vi "engine mappings UI.vi"() -> ()   [LabVIEW 2014, in "PL Framework Configuration Tool.lvlib" / "Engine Mappings.lvclass"]
uses:
  Engine Mappings.lvclass
  <vilib>/NI/Configuration Framework/Node/NodeRef.ctl
  <vilib>/NI/Configuration Framework/Node/NISE_CEF_Node.lvclass
  <vilib>/NI/AMC/Message Queue.ctl
  <vilib>/NI/AMC/Message.ctl
  <vilib>/NI/Tools/Keyed Array/KeyedArray.ctl
  <vilib>/NI/Configuration Framework/Node/UserEventRef.ctl
  <vilib>/NI/Configuration Framework/Controls/EventCluster.ctl
  <vilib>/NI/DCAF UI Toolkit/Controls/Move One Right.ctl
  <vilib>/NI/DCAF UI Toolkit/Controls/Move One Left.ctl
  <vilib>/NI/DCAF UI Toolkit/Controls/Export.ctl
  <vilib>/NI/Configuration Framework/Node/RefreshUIEvent.ctl
  <vilib>/NI/Configuration Framework/Node/CacheState.ctl
  <vilib>/NI/Configuration Framework/Node/StopEvent.ctl
  <vilib>/NI/Configuration Framework/Node/NodeChangeEvent.ctl
  subVIs/Mapping.ctl
  <vilib>/Utility/miscctls.llb/LVPositionTypeDef.ctl
  <vilib>/NI/Configuration Framework/serializable configuration/NISE_CEF_serializable configuration.lvclass/NISE_CEF_serializable configuration.ctl
  <vilib>/NI/Tag Bus/tag/tag descriptor.lvclass/tag descriptor.ctl
  <vilib>/NI/Tag Bus Module Framework/channel/channel classification.ctl
  <vilib>/NI/Configuration Framework/serializable configuration/get alias.vi
  <vilib>/Utility/LVClass/Get LV Class Name.vi
  <vilib>/NI/Configuration Framework/error generator/NISE_error generator.vi
  <vilib>/NI/Tag Bus Module Framework/module configuration/TBM module configuration.lvclass
  <vilib>/NI/Module Execution Interface/Engine Configuration/engine configuration.lvclass
  <vilib>/NI/Tag Bus/tag/tag descriptor.lvclass
  Engine Parent/Engine Parent Editor Node.lvclass
  Robust CSV/Robust CSV.lvlib
  <vilib>/NI/Configuration Framework/serializable configuration/NISE_CEF_serializable configuration.lvclass
  <vilib>/NI/Tag Bus Module Framework/channel/TBM channel.lvclass
  Utilities/GraphViz Vizualizations/GraphViz Mapping Visualizer.lvlib
  <vilib>/NI/DCAF UI Toolkit/Controls/DCAF UI Elements.lvlib
  <vilib>/NI/Tools/Keyed Array/Tools_KeyedArray.lvlib
  <vilib>/NI/AMC/AMC.lvlib
  <vilib>/NI/Configuration Framework/NISE_CEF_TreeControl.lvlib
panel:
  in  "Tab Control":T1(tab)
  in  "Show Mappings":T2
  in  "channels":i32(listbox)
  in  "Tags":i32(listbox)
  in  "map":T3
  in  "unmap":T4
  in  "export CSV":T5
  in  "Mappings":i32(listbox)
  out "Writer Channel":string
  out "channels reading tag to outout":i32(listbox)
  out "channels from input":i32(listbox)
  in  "outputs":i32(listbox)
  in  "method selection":enum32{"Inputs and Outputs", "Processing"}(radio)
  in  "inputs":i32(listbox)
  in  "Module to View":u16(ring)
  in  "attempt mapping":bool
  in  "Module 1 Filter":string
  in  "Module 2 Filter":string
  in  "Module 2 Channels":i32[](listbox)
  in  "Module 1 Channels":i32[](listbox)
  in  "Module 2":u16(ring)
  in  "Module 1":u16(ring)
  in  "main queue":T6
  in  "node ref":T7
  in  "user event":T8
  in  "node change":T9
  in  "stop event":T10
  in  "cache state":T11
  in  "refresh UI":T12
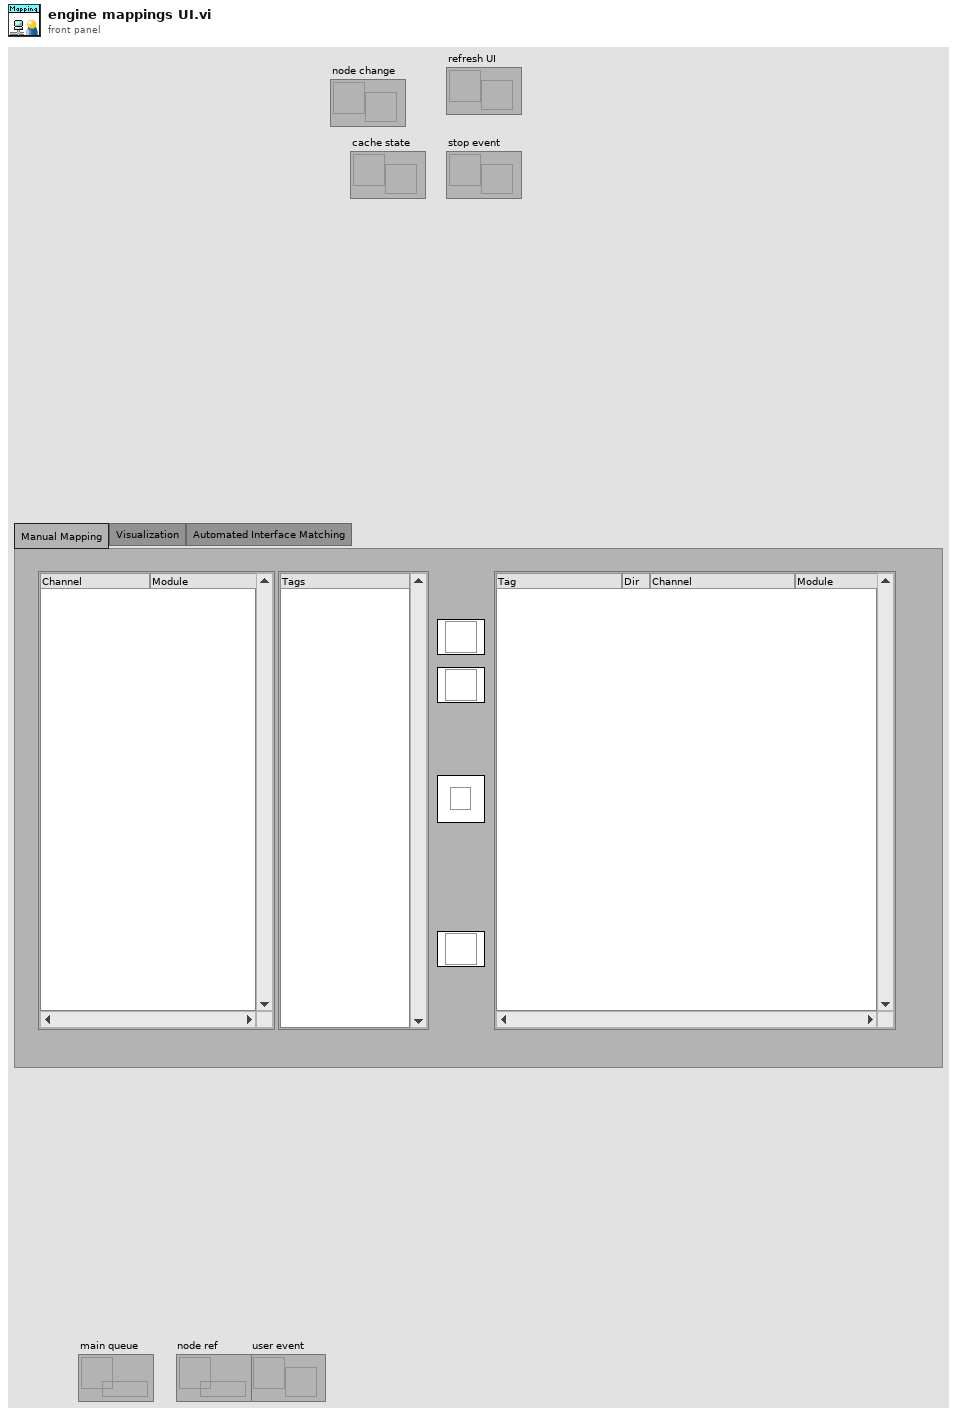
[diagram p1: front panel]
types:
  T1 = enum32{"Manual Mapping", "Visualization", "Automated Interface Matching"}
  T2 = typedef "Mapping.ctl" = bool
  T3 = typedef "DCAF UI Elements.lvlib/Move One Right.ctl" = bool
  T4 = typedef "DCAF UI Elements.lvlib/Move One Left.ctl" = bool
  T5 = typedef "DCAF UI Elements.lvlib/Export.ctl" = bool
  T6 = typedef "AMC.lvlib/Message Queue.ctl" = refnum<queue>
  T7 = typedef "NISE_CEF_Node.lvclass/NodeRef.ctl" = refnum<data-value>
  T8 = typedef "NISE_CEF_Node.lvclass/UserEventRef.ctl" = refnum<user-event>
  T9 = typedef "NISE_CEF_Node.lvclass/NodeChangeEvent.ctl" = refnum<user-event>
  T10 = typedef "NISE_CEF_Node.lvclass/StopEvent.ctl" = refnum<user-event>
  T11 = typedef "NISE_CEF_Node.lvclass/CacheState.ctl" = refnum<user-event>
  T12 = typedef "NISE_CEF_Node.lvclass/RefreshUIEvent.ctl" = refnum<user-event>
  T13 = typedef "LVPositionTypeDef.ctl" = cluster{"Left":i32, "Top":i32}
  T14 = typedef "TBM channel.lvclass/channel classification.ctl" = enum16{"input data", "output data", "processing parameter", "processing result"}
  T15 = typedef "engine configuration.lvclass/unique channel identifier.ctl" = cluster{"channel":string, "module ID":string}
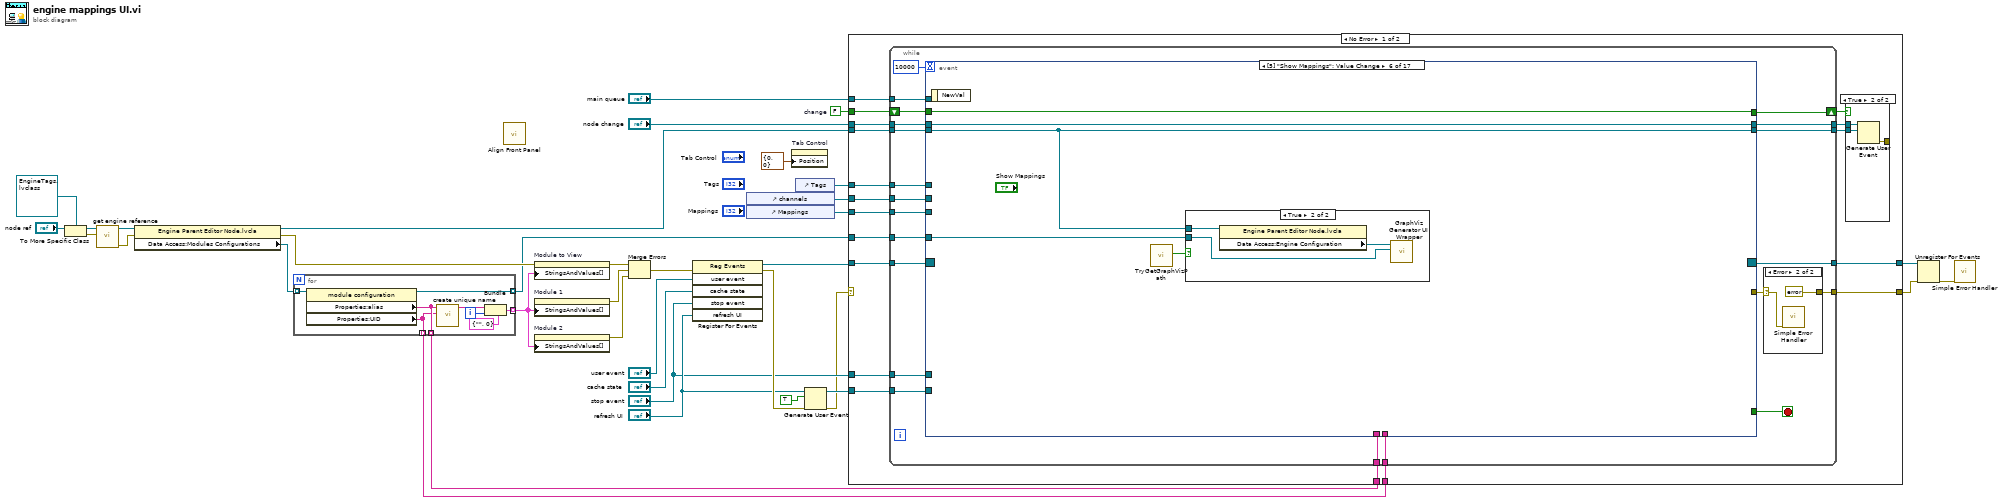
[diagram p0: block diagram]
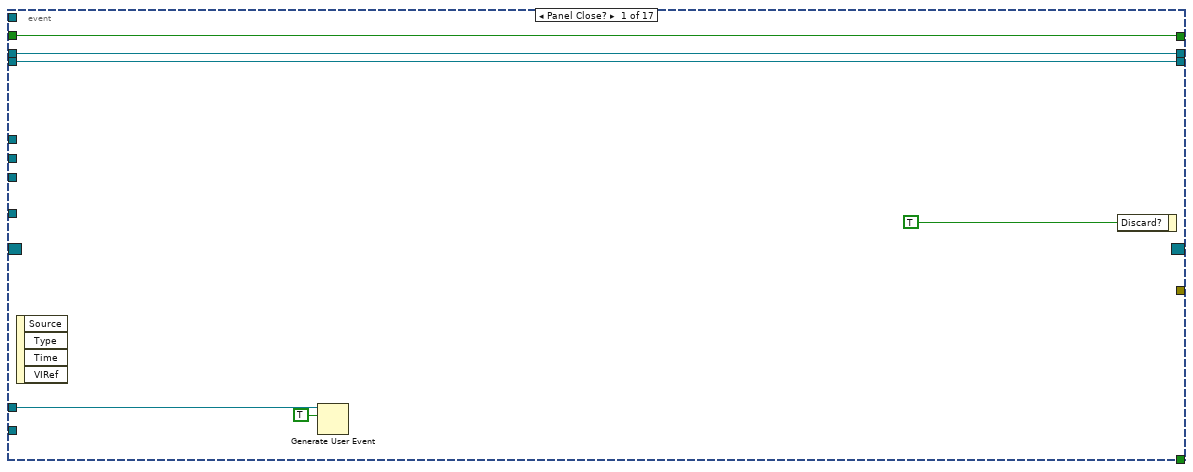
[diagram p4: hidden frame]
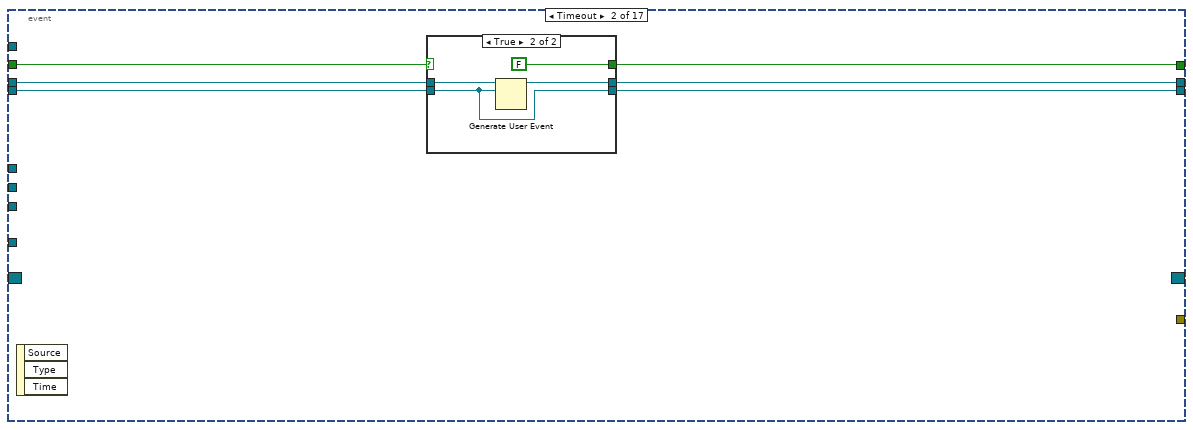
[diagram p5: hidden frame]
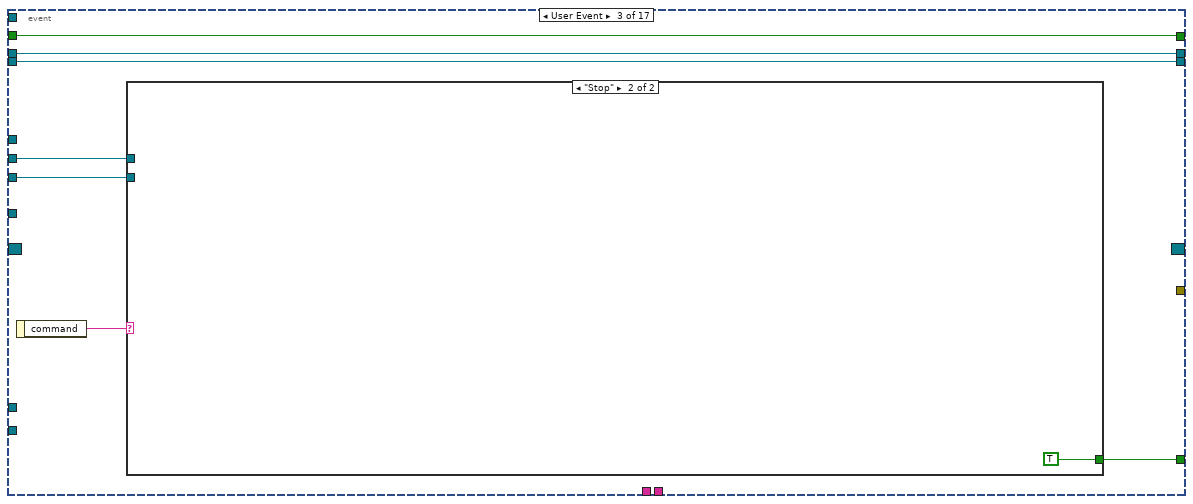
[diagram p7: hidden frame]
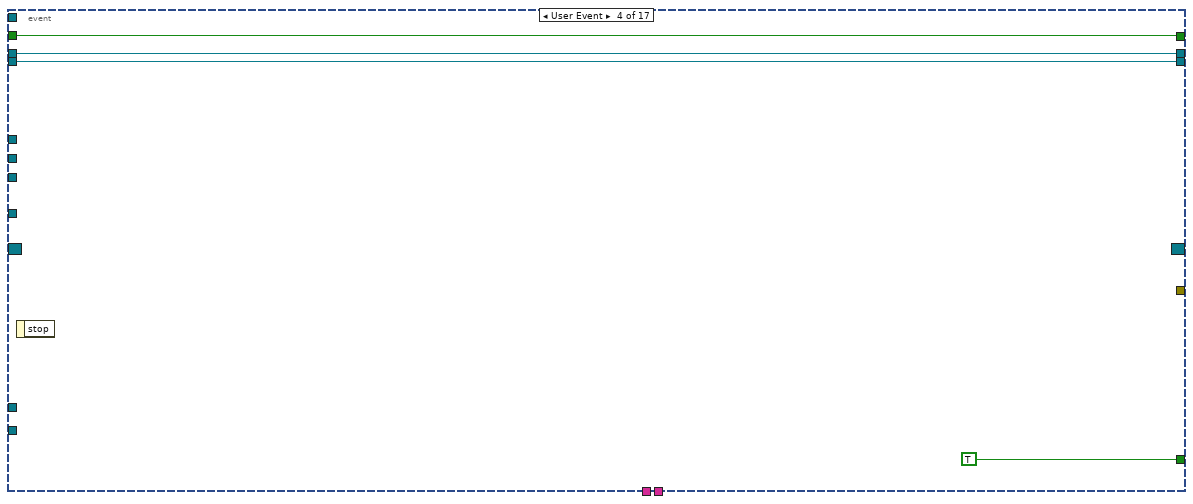
[diagram p9: hidden frame]
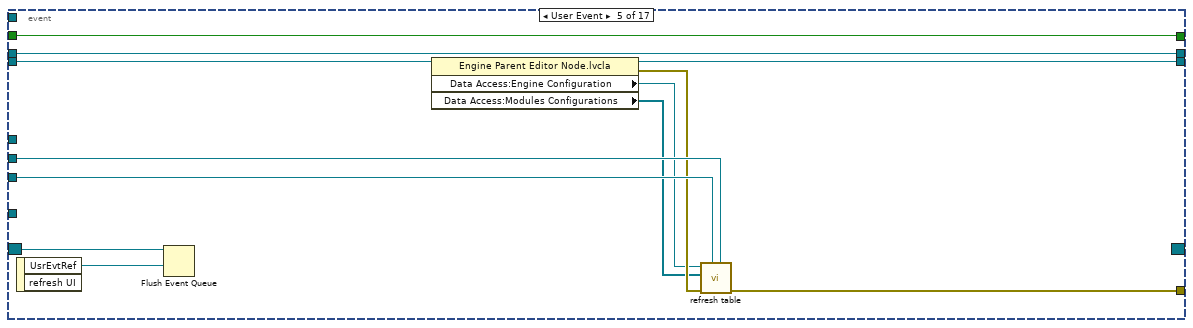
[diagram p10: hidden frame]
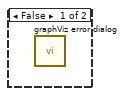
[diagram p11: hidden frame]
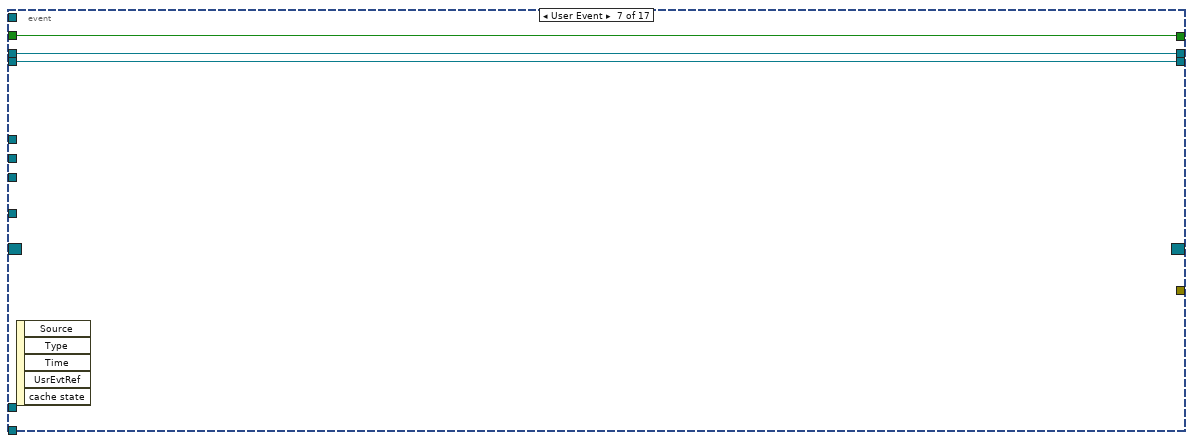
[diagram p12: hidden frame]
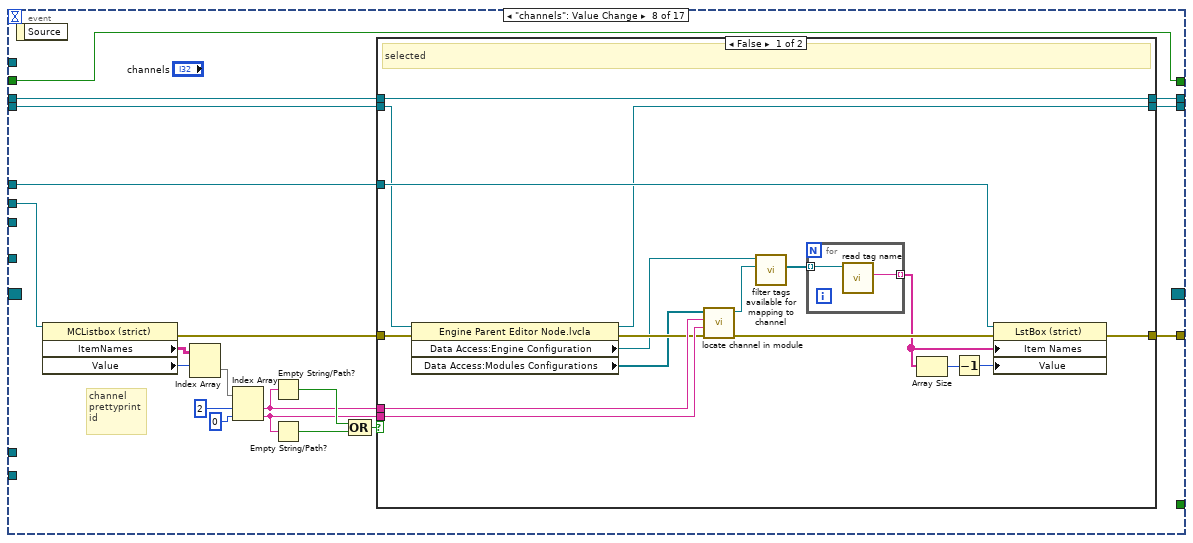
[diagram p13: hidden frame]
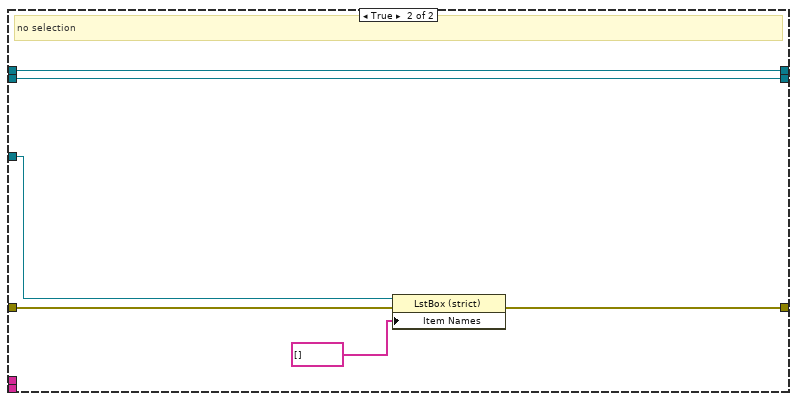
[diagram p14: hidden frame]
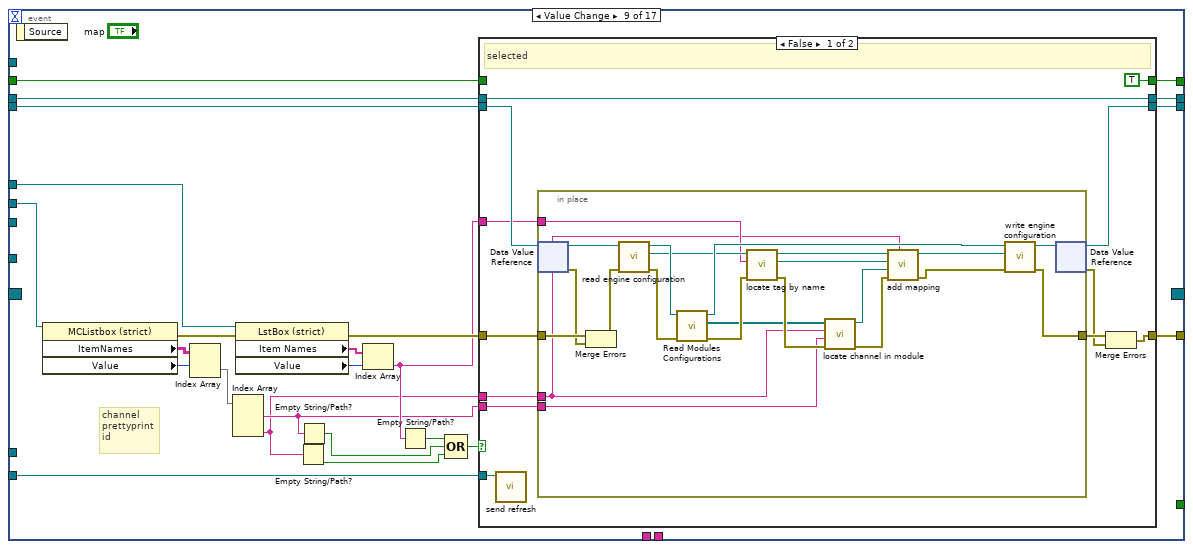
[diagram p15: hidden frame]
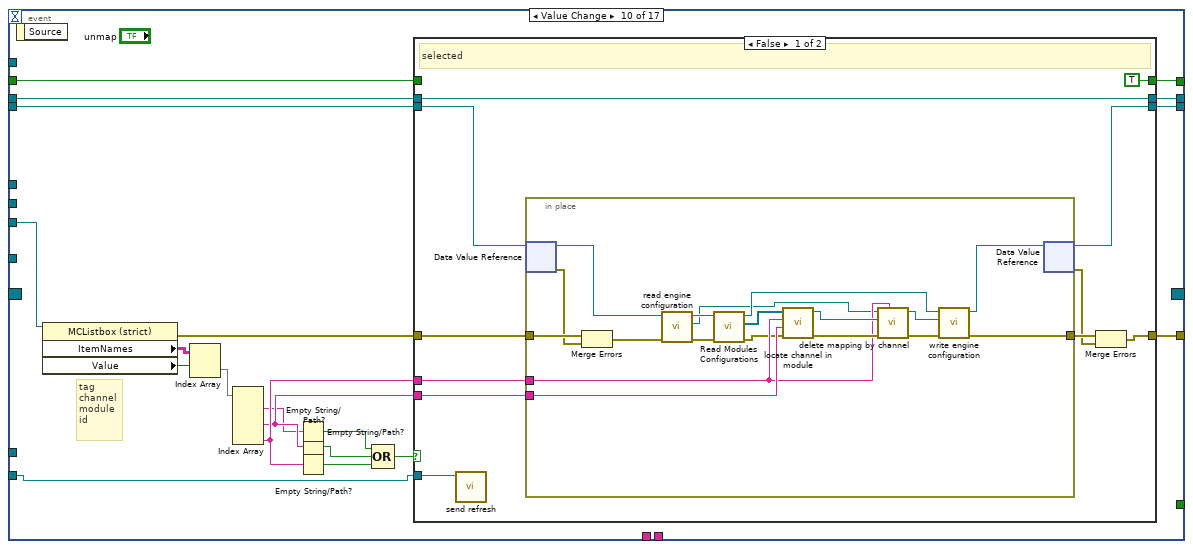
[diagram p17: hidden frame]
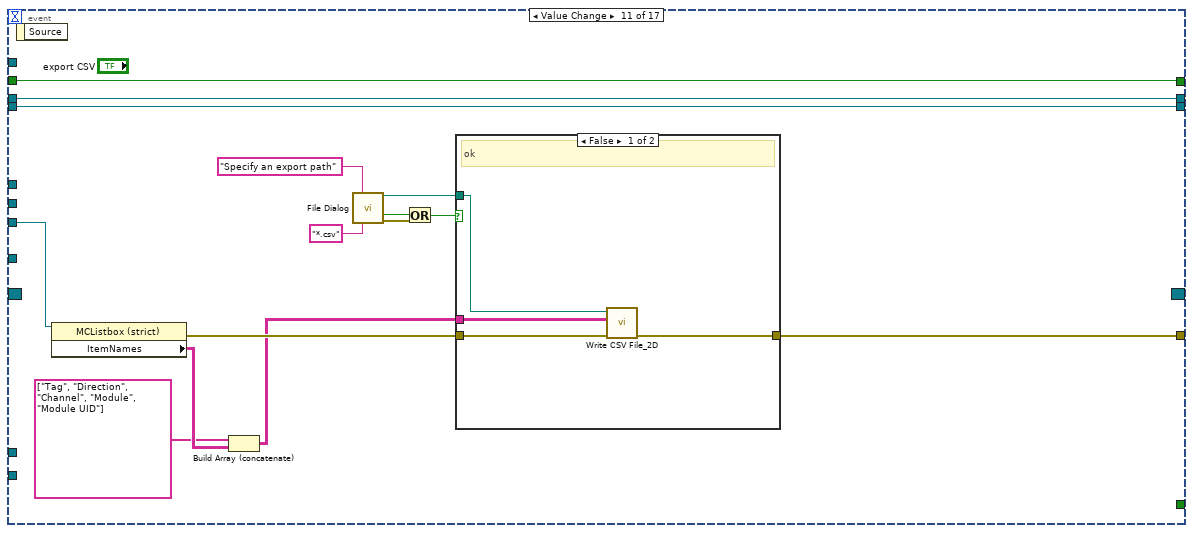
[diagram p19: hidden frame]
diagram:
  w1 = FALSE  # change
  n1 = To More Specific Class(target class=refnum<data-value> refnum ("data value reference"), reference="node ref") -> (specific class reference=w22:refnum<data-value>, error out=w23:errorcluster)  [unwired: 1 in]
  n2 = call "get engine reference.vi"("error in"=w23, "engine mappings"=w22) -> ("error out"=w25:errorcluster, "engine reference"=w17:refnum<data-value>)  [unwired: 8 in]
  n3 = property class="Engine Parent Editor Node.lvcla"(reference=w17, error in=w25) -> (reference out=w16:refnum<data-value>, error out=w15:errorcluster, "Data Access:Modules Configurations"=w14:refnum<class "TBM module configuration.lvclass">[])
  n4 = for {
    tunnel: w14 -> [w44] mode=indexing
    tunnel: [w43] -> w13 mode=indexing
    tunnel: [w42] -> w12 mode=indexing
    tunnel: [w40] -> w11 mode=indexing
    tunnel: [w37] -> w2 mode=indexing
    i -> [w38]
    n5 = property class="module configuration"(reference=w44) -> (reference out=w37:refnum<class "TBM module configuration.lvclass">, "Properties:alias"=w43:string, "Properties:UID"=w42:string)  [unwired: 1 in, 1 out]
    n6 = call "create unique name.vi"("UID"=w42, "alias"=w43) -> ("unique ring name"=w39:string)  [unwired: 9 in]
    n7 = Bundle(cluster=cluster{"String":string, "Value":u16} {"String"="", "Value"=0}, "String"=w39, "Value"=w38) -> (w40:cluster{"String":string, "Value":u16})
  }
  n8 = call <vilib>:"Align Front Panel.vi"() -> ()  [unwired: 10 in, 2 out]
  n9 = property on="Module to View" class="Ring (strict)"(error in=w15, "StringsAndValues[]"=w11) -> (error out=w8:errorcluster)  [unwired: 1 in, 1 out]
  n10 = property on="Module 1" class="Ring (strict)"("StringsAndValues[]"=w11) -> (error out=w7:errorcluster)  [unwired: 2 in, 1 out]
  n11 = property on="Module 2" class="Ring (strict)"("StringsAndValues[]"=w11) -> (error out=w6:errorcluster)  [unwired: 2 in, 1 out]
  n12 = Merge Errors(w8, w7, w6) -> (w5:errorcluster)
  n13 = register-events(error in=w5, "user event", "cache state", "stop event", "refresh UI") -> (reference out=w35:refnum<event-registration>, error out=w32:errorcluster)  [unwired: 1 in]
  n14 = control-ref of="channels"() -> (w27:refnum<vi>)
  n15 = control-ref of="Mappings"() -> (w26:refnum<vi>)
  n16 = property on="Tab Control" class="TabCtl (strict)"("Position"=T13 {"Left"=0, "Top"=0}) -> ()  [unwired: 2 in, 2 out]
  n17 = control-ref of="Tags"() -> (w28:refnum<vi>)
  n18 = Generate User Event(user event="refresh UI", event data cluster=TRUE ("event data"), error in=w32) -> (user event out=w29:T12, error out=w4:errorcluster)  [unwired: 1 in]
  n19 = case shown="No Error" w4 {
    selector: w4 -> [_ w653]
    tunnel: "main queue" -> [w62 _]
    tunnel: w35 -> [w61 w654]
    tunnel: [w60 w654] -> w34
    tunnel: [w59 w653] -> w33
    tunnel: w16 -> [w48 _]
    tunnel: w29 -> [w58 _]
    tunnel: w28 -> [w57 _]
    tunnel: w27 -> [w56 _]
    tunnel: w26 -> [w55 _]
    tunnel: "stop event" -> [w54 _]
    tunnel: "node change" -> [w52 _]
    tunnel: w2 -> [w51 _]
    tunnel: w13 -> [w50 _]
    tunnel: w12 -> [w49 _]
    tunnel: w1 -> [w45 _]
    frame No Error {
      n20 = while {
        tunnel: w62 -> [w86]
        tunnel: w61 -> [w85]
        tunnel: [w84] -> w60
        tunnel: w48 -> [w81]
        tunnel: w58 -> [w79]
        tunnel: w57 -> [w78]
        tunnel: w56 -> [w77]
        tunnel: w55 -> [w76]
        tunnel: w54 -> [w75]
        tunnel: [w82] -> w59
        shift-right: [w73] -> w53
        shift-left: w45 -> [w74]
        tunnel: w52 -> [w71]
        tunnel: w51 -> [w70]
        tunnel: w50 -> [w69]
        tunnel: w49 -> [w68]
        tunnel: [w67] -> w47
        tunnel: [w66] -> w46
        stop <- w83 stop-if-true
        n21 = event shown="[5] \"Show Mappings\": Value Change" {
          selector: w85 -> [_ _ _ _ w125 _ _ _ _ _ _ _ _ _ _ _ _]
          dyn-events: [_ _ _ _ _ _ _ _ _ _ _ _ _ _ _ _ _] -> w84
          timeout: 10000 -> [_ _ _ _ _ _ _ _ _ _ _ _ _ _ _ _ _]
          tunnel: w86 -> [_ _ _ _ _ _ _ _ _ _ _ _ _ _ _ _ _]
          tunnel: [_ _ w115 TRUE _ _ _ _ _ _ _ _ _ _ _ _ _] -> w83
          tunnel: [_ _ _ _ w132 _ _ w154 w198 w263 w308 _ w385 w448 w515 w539 w560] -> w80
          tunnel: w81 -> [w90 w97 w109 w117 w122 w135 w141 w151 w193 w255 w303 w324 w388 w451 w512 w535 w561]
          tunnel: w79 -> [_ _ _ _ _ _ _ _ w197 w262 _ _ _ _ _ _ _]
          tunnel: w78 -> [_ _ _ _ _ _ _ w152 w211 _ _ _ _ _ _ _ _]
          tunnel: w77 -> [_ _ w113 _ w131 _ _ w161 w209 _ _ _ _ _ _ _ _]
          tunnel: w76 -> [_ _ w112 _ w130 _ _ _ _ w261 w317 _ _ _ _ _ _]
          tunnel: w75 -> [w94 _ _ _ _ _ _ _ _ _ _ _ _ _ _ _ _]
          tunnel: w74 -> [w92 w101 w111 w119 w126 w137 w143 w150 w192 w253 w305 w335 w403 w465 w525 w548 w558]
          tunnel: [w92 w100 w111 w119 w126 w137 w143 w150 w191 w254 w305 w335 w403 w465 w525 w548 w586] -> w73
          tunnel: w71 -> [w91 w99 w110 w118 w123 w133 w142 w144 w189 w250 w304 w325 w382 w444 w513 w536 w559]
          tunnel: w70 -> [_ _ _ _ _ w136 _ _ _ _ _ w334 w394 w457 w520 w543 w568]
          tunnel: w69 -> [_ _ _ _ _ _ _ _ _ _ _ _ w384 w447 _ _ _]
          tunnel: w68 -> [_ _ _ _ _ _ _ _ _ _ _ _ w383 w446 _ _ _]
          tunnel: [w90 w96 w109 w117 w121 w135 w141 w146 w188 w252 w303 w323 w381 w443 w512 w535 w561] -> w67
          tunnel: [w91 w98 w110 w118 w123 w133 w142 w145 w190 w251 w304 w325 w382 w444 w513 w536 w559] -> w66
          event Panel Close? {
            n22 = event-data() -> ()  [unwired: 1 in, 4 out]
            n23 = Generate User Event(user event=w94, event data cluster=TRUE ("event data")) -> ()  [unwired: 2 in, 2 out]
            n24 = event-data("Discard?"=TRUE) -> ()  [unwired: 1 in, 1 out]
          }
          event Timeout {
            n25 = event-data() -> ()  [unwired: 1 in, 3 out]
            n26 = case shown="True" w101 {
              selector: w101 -> [w104 _]
              tunnel: [w104 FALSE] -> w100
              tunnel: w99 -> [w103 w107]
              tunnel: w97 -> [w102 w105]
              tunnel: [w103 w106] -> w98
              tunnel: [w102 w105] -> w96
              frame False {
              }
              frame True {
                n27 = Generate User Event(user event=w107, event data cluster=w105) -> (user event out=w106:T9)  [unwired: 2 in, 1 out]
              }
            }
          }
          event User Event {
            n28 = event-data() -> ("command"=w114:string)  [unwired: 1 in]
            n29 = case shown="\"Stop\"" w114 {
              tunnel: [_ TRUE] -> w115
              tunnel: w113 -> [_ _]
              tunnel: w112 -> [_ _]
              frame Default {
              }
              frame "Stop" {
              }
            }
          }
          event User Event {
            n30 = event-data() -> ()  [unwired: 1 in, 1 out]
          }
          event User Event {
            n31 = event-data() -> ("UsrEvtRef"=w124:refnum<user-event>)  [unwired: 1 in, 1 out]
            n32 = Flush Event Queue(0:w125, 2:w124) -> ()  [unwired: 4 in, 3 out]
            n33 = property class="Engine Parent Editor Node.lvcla"(reference=w122) -> (reference out=w121:refnum<data-value>, error out=w129:errorcluster, "Data Access:Engine Configuration"=w128:refnum<class "engine configuration.lvclass">, "Data Access:Modules Configurations"=w127:refnum<class "TBM module configuration.lvclass">[])  [unwired: 1 in]
            n34 = call "refresh table.vi"("channels ref"=w131, "Mappings"=w130, "error in"=w129, "Modules Configurations"=w127, "engine configuration in"=w128) -> ("error out"=w132:errorcluster)  [unwired: 6 in]
          }
          event Value Change {
            n35 = event-data() -> ()  [unwired: 1 in, 1 out]
            n36 = call "TryGetGraphVizPath.vi"() -> ("Found?"=w134:bool)  [unwired: 10 in, 1 out]
            n37 = case shown="True" w134 {
              tunnel: w136 -> [_ w140]
              tunnel: w135 -> [_ w139]
              frame False {
                n38 = call "graphViz error dialog.vi"() -> ()  [unwired: 12 in]
              }
              frame True {
                n39 = property class="Engine Parent Editor Node.lvcla"(reference=w139) -> ("Data Access:Engine Configuration"=w138:refnum<class "engine configuration.lvclass">)  [unwired: 1 in, 2 out]
                n40 = call "GraphViz Generator UI Wrapper.vi"("Modules Configurations"=w140, "engine configuration in"=w138) -> ()  [unwired: 10 in]
              }
            }
          }
          event User Event {
            n41 = event-data() -> ()  [unwired: 1 in, 5 out]
          }
          event "channels": Value Change {
            # "channel\nprettyprint\nid"
            n42 = event-data() -> ()  [unwired: 1 in, 1 out]
            n43 = property class="MCListbox (strict)"(reference=w161) -> (error out=w162:errorcluster, "ItemNames"=w159:string[][], "Value"=w160:i32)  [unwired: 1 in, 1 out]
            n44 = Index Array(array=w159, index (row)=w160) -> (element=w158:string[])  [unwired: 1 in]
            n45 = Index Array(array=w158, index #1=2 ("index"), index #2=0 ("index")) -> (element #1=w147:string, element #2=w153:string)
            n46 = Empty String/Path?(string/path=w147) -> (empty?=w157:bool)
            n47 = Empty String/Path?(string/path=w153) -> (empty?=w156:bool)
            n48 = Compound Arithmetic op=OR(w157, w156) -> (w155:bool)
            n49 = case shown="False" w155 {
              tunnel: w162 -> [w179 w187]
              tunnel: [w174 w186] -> w154
              tunnel: w153 -> [w178 _]
              tunnel: w147 -> [w177 _]
              tunnel: w152 -> [w175 w185]
              tunnel: w151 -> [w168 w183]
              tunnel: [w164 w183] -> w146
              tunnel: [w163 w182] -> w145
              tunnel: w144 -> [w163 w182]
              frame False {
                # "selected"
                n50 = property class="Engine Parent Editor Node.lvcla"(reference=w168, error in=w179) -> (reference out=w164:refnum<data-value>, error out=w167:errorcluster, "Data Access:Engine Configuration"=w165:refnum<class "engine configuration.lvclass">, "Data Access:Modules Configurations"=w166:refnum<class "TBM module configuration.lvclass">[])
                n51 = call "locate channel in module.vi"("error in"=w167, "channel name"=w178, "instance id"=w177, "Modules Configurations"=w166) -> ("error out"=w173:errorcluster, "channel"=w176:refnum<class "TBM channel.lvclass">)  [unwired: 6 in]
                n52 = call-dynamic "filter tags available for mapping to channel.vi"("channel to map to"=w176, "engine configuration in"=w165) -> ("filtered tags"=w172:refnum<class "tag descriptor.lvclass">[])  [unwired: 8 in, 1 out]
                n53 = for {
                  tunnel: w172 -> [w181] mode=indexing
                  tunnel: [w180] -> w171 mode=indexing
                  n54 = call <vilib>:"read tag name.vi"("system tag in"=w181) -> ("name"=w180:string)  [unwired: 8 in, 2 out]
                }
                n55 = Array Size(array=w171) -> (size(s)=w170:i32)
                n56 = Decrement(x=w170) -> (x-1=w169:i32)
                n57 = property class="LstBox (strict)"(reference=w175, error in=w173, "Item Names"=w171, "Value"=w169) -> (error out=w174:errorcluster)  [unwired: 1 out]
              }
              frame True {
                # "no selection"
                n58 = property class="LstBox (strict)"(reference=w185, error in=w187, "Item Names"=string[] []) -> (error out=w186:errorcluster)  [unwired: 1 out]
              }
            }
          }
          event Value Change {
            # "channel\nprettyprint\nid"
            n59 = event-data() -> ()  [unwired: 1 in, 1 out]
            n60 = property class="MCListbox (strict)"(reference=w209) -> (error out=w210:errorcluster, "ItemNames"=w207:string[][], "Value"=w208:i32)  [unwired: 1 in, 1 out]
            n61 = Index Array(array=w207, index (row)=w208) -> (element=w204:string[])  [unwired: 1 in]
            n62 = Index Array(array=w204) -> (element #1=w195:string, element #3=w194:string)  [unwired: 3 in, 1 out]
            n63 = property class="LstBox (strict)"(reference=w211, error in=w210) -> (error out=w199:errorcluster, "Item Names"=w206:string[], "Value"=w205:i32)  [unwired: 1 out]
            n64 = Empty String/Path?(string/path=w194) -> (empty?=w203:bool)
            n65 = Empty String/Path?(string/path=w195) -> (empty?=w202:bool)
            n66 = Index Array(array=w206, index=w205) -> (element=w196:string)
            n67 = Empty String/Path?(string/path=w196) -> (empty?=w201:bool)
            n68 = Compound Arithmetic op=OR(w201, w202, w203) -> (w200:bool)
            n69 = case shown="False" w200 {
              tunnel: w199 -> [w223 w249]
              tunnel: [w221 w249] -> w198
              tunnel: w197 -> [w214 _]
              tunnel: w196 -> [w218 _]
              tunnel: w195 -> [w216 _]
              tunnel: w194 -> [w217 _]
              tunnel: w193 -> [w219 w247]
              tunnel: w192 -> [_ w248]
              tunnel: [TRUE ("change") w248] -> w191
              tunnel: [w213 w246] -> w190
              tunnel: w189 -> [w213 w246]
              tunnel: [w212 w247] -> w188
              frame False {
                # "selected"
                n70 = call "send refresh.vi"("refresh UI"=w214) -> ()  [unwired: 11 in]
                n71 = in-place {
                  in-place-border: w223 -> [w245]
                  in-place-border: [w240] -> w222
                  in-place-border: w218 -> [w234]
                  in-place-border: w217 -> [w224]
                  in-place-border: w216 -> [w230]
                  n72 = in-place-dvr #1(w219) -> (w237:refnum<class "Engine Parent Editor Node.lvclass">, w244:errorcluster)
                  n73 = Merge Errors(w245, w244) -> (w243:errorcluster)
                  n74 = call "read engine configuration.vi"("error in"=w243, "Engine Parent Editor Node in"=w237) -> ("error out"=w242:errorcluster, "engine configuration"=w236:refnum<class "engine configuration.lvclass">, "Engine Parent Editor Node out"=w241:refnum<class "Engine Parent Editor Node.lvclass">)  [unwired: 7 in]
                  n75 = call "Read Modules Configurations.vi"("error in"=w242, "Engine Parent in"=w241) -> ("error out"=w233:errorcluster, "Component Configurations"=w231:refnum<class "TBM module configuration.lvclass">[], "Engine Parent out"=w238:refnum<class "Engine Parent Editor Node.lvclass">)  [unwired: 7 in]
                  n76 = call <vilib>:"locate tag by name.vi"("error in"=w233, "tag name"=w234, "engine configuration in"=w236) -> ("error out"=w232:errorcluster, "tag descriptor"=w228:refnum<class "tag descriptor.lvclass">, "engine configuration out"=w235:refnum<class "engine configuration.lvclass">)  [unwired: 6 in]
                  n77 = call "locate channel in module.vi"("error in"=w232, "channel name"=w230, "instance id"=w224, "Modules Configurations"=w231) -> ("error out"=w227:errorcluster, "channel"=w229:refnum<class "TBM channel.lvclass">)  [unwired: 6 in]
                  n78 = call-dynamic "add mapping.vi"("owner ID"=w224, "error in"=w227, "channel"=w229, "tag descriptor"=w228, "engine configuration"=w235) -> ("error out"=w226:errorcluster, "engine configuration out"=w225:refnum<class "engine configuration.lvclass">)  [unwired: 5 in]
                  n79 = call "write engine configuration.vi"("error in"=w226, "engine configuration"=w225, "Engine Parent Editor Node in"=w238) -> ("error out"=w240:errorcluster, "Engine Parent Editor Node out"=w239:refnum<class "Engine Parent Editor Node.lvclass">)  [unwired: 7 in]
                  n80 = in-place-dvr #1(w239) -> (w212:refnum<data-value>, w220:errorcluster)
                }
                n81 = Merge Errors(w222, w220) -> (w221:errorcluster)
              }
              frame True {
                # "no selection"
              }
            }
          }
          event Value Change {
            # "tag\nchannel\nmodule\nid"
            n82 = event-data() -> ()  [unwired: 1 in, 1 out]
            n83 = property class="MCListbox (strict)"(reference=w261) -> (error out=w269:errorcluster, "ItemNames"=w267:string[][], "Value"=w268:i32)  [unwired: 1 in, 1 out]
            n84 = Index Array(array=w267, index (row)=w268) -> (element=w266:string[])  [unwired: 1 in]
            n85 = Index Array(array=w266) -> (element #1=w256:string, element #3=w257:string, element #5=w260:string)  [unwired: 5 in, 2 out]
            n86 = Empty String/Path?(string/path=w256) -> (empty?=w258:bool)
            n87 = Empty String/Path?(string/path=w257) -> (empty?=w259:bool)
            n88 = Empty String/Path?(string/path=w260) -> (empty?=w265:bool)
            n89 = Compound Arithmetic op=OR(w258, w259, w265) -> (w264:bool)
            n90 = case shown="False" w264 {
              tunnel: w269 -> [w280 w302]
              tunnel: [w275 w302] -> w263
              tunnel: w262 -> [w273 _]
              tunnel: w257 -> [w279 _]
              tunnel: w260 -> [w278 _]
              tunnel: w255 -> [w276 w300]
              tunnel: [TRUE ("change") w301] -> w254
              tunnel: w253 -> [_ w301]
              tunnel: [w271 w300] -> w252
              tunnel: [w270 w299] -> w251
              tunnel: w250 -> [w270 w299]
              frame False {
                # "selected"
                n91 = call "send refresh.vi"("refresh UI"=w273) -> ()  [unwired: 11 in]
                n92 = in-place {
                  in-place-border: w280 -> [w298]
                  in-place-border: w279 -> [w297]
                  in-place-border: w278 -> [w294]
                  in-place-border: [w286] -> w277
                  n93 = in-place-dvr #2(w276) -> (w282:refnum<class "Engine Parent Editor Node.lvclass">, w293:errorcluster)
                  n94 = Merge Errors(w298, w293) -> (w292:errorcluster)
                  n95 = call "read engine configuration.vi"("error in"=w292, "Engine Parent Editor Node in"=w282) -> ("error out"=w291:errorcluster, "engine configuration"=w281:refnum<class "engine configuration.lvclass">, "Engine Parent Editor Node out"=w290:refnum<class "Engine Parent Editor Node.lvclass">)  [unwired: 7 in]
                  n96 = call "Read Modules Configurations.vi"("error in"=w291, "Engine Parent in"=w290) -> ("error out"=w289:errorcluster, "Component Configurations"=w288:refnum<class "TBM module configuration.lvclass">[], "Engine Parent out"=w283:refnum<class "Engine Parent Editor Node.lvclass">)  [unwired: 7 in]
                  n97 = call "locate channel in module.vi"("error in"=w289, "channel name"=w297, "instance id"=w294, "Modules Configurations"=w288) -> ("error out"=w296:errorcluster, "channel"=w295:refnum<class "TBM channel.lvclass">)  [unwired: 6 in]
                  n98 = call <vilib>:"delete mapping by channel.vi"("owner ID"=w294, "error in"=w296, "channel"=w295, "engine configuration in"=w281) -> ("error out"=w287:errorcluster, "engine configuration out"=w284:refnum<class "engine configuration.lvclass">)  [unwired: 6 in]
                  n99 = call "write engine configuration.vi"("error in"=w287, "engine configuration"=w284, "Engine Parent Editor Node in"=w283) -> ("error out"=w286:errorcluster, "Engine Parent Editor Node out"=w285:refnum<class "Engine Parent Editor Node.lvclass">)  [unwired: 7 in]
                  n100 = in-place-dvr #2(w285) -> (w271:refnum<data-value>, w274:errorcluster)
                }
                n101 = Merge Errors(w277, w274) -> (w275:errorcluster)
              }
              frame True {
                # "no selection"
              }
            }
          }
          event Value Change {
            n102 = event-data() -> ()  [unwired: 1 in, 1 out]
            n103 = property class="MCListbox (strict)"(reference=w317) -> (error out=w307:errorcluster, "ItemNames"=w316:string[][])  [unwired: 1 in, 1 out]
            n104 = Build Array (concatenate)(string[] ["Tag", "Direction", "Channel", "Module", "Module UID"], w316) -> (w306:string[][])
            n105 = call "File Dialog"("prompt"="Specify an export path", "pattern (all files)"="*.csv") -> ("selected path"=w309:path, "cancelled"=w311:bool, "error out"=w312:errorcluster)  [unwired: 10 in, 1 out]
            n106 = Or(x=w311, y=w312) -> (x .or. y?=w310:bool)
            n107 = case shown="False" w310 {
              tunnel: w309 -> [w321 _]
              tunnel: [w318 w322] -> w308
              tunnel: w307 -> [w320 w322]
              tunnel: w306 -> [w319 _]
              frame False {
                # "ok"
                n108 = call "Write CSV File_2D.vi"("error in (no error)"=w320, "2D array"=w319, "file path in"=w321) -> ("error out"=w318:errorcluster)  [unwired: 7 in, 1 out]
              }
              frame True {
                # "error"
              }
            }
          }
          event "Module to View", "method selection": Value Change {
            n109 = event-data() -> ()  [unwired: 1 in, 1 out]
            n110 = Index Array(array=w334, index="Module to View") -> (element=w332:refnum<class "TBM module configuration.lvclass">)
            n111 = call <vilib>:"Read UID.vi"("configuration in"=w332) -> ("error out"=w330:errorcluster, "instance id"=w326:string, "configuration out"=w328:refnum<class "TBM module configuration.lvclass">)  [unwired: 8 in]
            n112 = Empty String/Path?(string/path=w326) -> (empty?=w331:bool)
            n113 = Or(x=w331, y=w330) -> (x .or. y?=w329:bool)
            n114 = case shown="False" w329 {
              tunnel: w328 -> [w352 _]
              tunnel: "method selection" -> [w351 _]
              tunnel: w326 -> [w342 _]
              tunnel: w324 -> [w345 w379]
              tunnel: [w336 w379] -> w323
              frame False {
                n115 = case shown="\"Inputs and Outputs\"" w351 {
                  tunnel: [channel_classification."input data" ("channel classification") channel_classification."processing result" ("channel classification")] -> w350
                  tunnel: [channel_classification."output data" ("channel classification") channel_classification."processing parameter" ("channel classification")] -> w349
                  frame "Inputs and Outputs" {
                  }
                  frame "Processing" {
                  }
                }
                n116 = property class="Engine Parent Editor Node.lvcla"(reference=w345) -> (reference out=w336:refnum<data-value>, "Data Access:Engine Configuration"=w340:refnum<class "engine configuration.lvclass">)  [unwired: 1 in, 1 out]
                n117 = call-dynamic "get channels.vi"("module configuration in"=w352) -> ("channels"=w346:refnum<class "TBM channel.lvclass">[])  [unwired: 9 in, 1 out]
                n118 = Build Array(w350) -> (w348:T14[])
                n119 = Build Array(w349) -> (w347:T14[])
                n120 = call <vilib>:"filter channels by classification.vi"("allowed classifications"=w348, "channels in"=w346) -> ("channels out"=w341:refnum<class "TBM channel.lvclass">[])  [unwired: 9 in]
                n121 = call <vilib>:"filter channels by classification.vi"("allowed classifications"=w347, "channels in"=w346) -> ("channels out"=w344:refnum<class "TBM channel.lvclass">[])  [unwired: 9 in]
                n122 = Sort 1D Array(array=w341) -> (sorted array=w337:refnum<class "TBM channel.lvclass">[])
                n123 = Sort 1D Array(array=w344) -> (sorted array=w338:refnum<class "TBM channel.lvclass">[])
                n124 = for {
                  tunnel: w337 -> [w362] mode=indexing
                  tunnel: w342 -> [w355]
                  tunnel: [w354] -> w339 mode=indexing
                  tunnel: w340 -> [w363]
                  n125 = call <vilib>:"find tag mapped to channel.vi"("owner"=w355, "channel"=w362, "engine configuration in"=w363) -> ("error out"=w361:errorcluster, "tag"=w360:refnum<class "tag descriptor.lvclass">)  [unwired: 6 in, 1 out]
                  n126 = call <vilib>:"read tag name.vi"("system tag in"=w362) -> ("name"=w353:string)  [unwired: 8 in, 2 out]
                  n127 = call <vilib>:"read tag name.vi"("error in"=w361, "system tag in"=w360) -> ("error out"=w359:errorcluster, "name"=w358:string)  [unwired: 7 in, 1 out]
                  n128 = Select(t="", s=w359, f=w358) -> (s? t:f=w356:string)
                  n129 = Build Array(w353, w356) -> (w354:string[])
                }
                n130 = for {
                  tunnel: w338 -> [w373] mode=indexing
                  tunnel: w342 -> [w365]
                  tunnel: [w364] -> w343 mode=indexing
                  tunnel: w340 -> [w374]
                  n131 = call <vilib>:"read tag name.vi"("system tag in"=w373) -> ("name"=w366:string)  [unwired: 8 in, 2 out]
                  n132 = call <vilib>:"find tag mapped to channel.vi"("owner"=w365, "channel"=w373, "engine configuration in"=w374) -> ("error out"=w372:errorcluster, "tag"=w371:refnum<class "tag descriptor.lvclass">)  [unwired: 6 in, 1 out]
                  n133 = call <vilib>:"read tag name.vi"("error in"=w372, "system tag in"=w371) -> ("error out"=w370:errorcluster, "name"=w369:string)  [unwired: 7 in, 1 out]
                  n134 = Select(t="", s=w370, f=w369) -> (s? t:f=w367:string)
                  n135 = Build Array(w367, w366) -> (w364:string[])
                }
                n136 = property on="inputs" class="MCListbox (strict)"("ItemNames"=w339) -> ()  [unwired: 2 in, 2 out]
                n137 = property on="outputs" class="MCListbox (strict)"("ItemNames"=w343) -> ()  [unwired: 2 in, 2 out]
              }
              frame True {
                n138 = One Button Dialog(message="No Module Selected") -> ()  [unwired: 1 in, 1 out]
              }
            }
          }
          event "inputs": Value Change {
            w399 = 0  # chan column
            n139 = event-data() -> ("CtlRef"=w402:refnum<vi>)  [unwired: 1 in]
            n140 = local read "Module to View"() -> (w398:u16)
            n141 = property class="Engine Parent Editor Node.lvcla"(reference=w388) -> (reference out=w381:refnum<data-value>, "Data Access:Engine Configuration"=w387:refnum<class "engine configuration.lvclass">)  [unwired: 1 in, 1 out]
            n142 = property class="MCListbox (strict)"(reference=w402) -> ("ItemNames"=w401:string[][])  [unwired: 1 in, 2 out]
            n143 = Index Array(array=w394, index=w398) -> (element=w397:refnum<class "TBM module configuration.lvclass">)
            n144 = call <vilib>:"Read UID.vi"("configuration in"=w397) -> ("error out"=w395:errorcluster, "instance id"=w386:string, "configuration out"=w390:refnum<class "TBM module configuration.lvclass">)  [unwired: 8 in]
            n145 = Empty String/Path?(string/path=w386) -> (empty?=w396:bool)
            n146 = Index Array(array=w401, index (row)="inputs", index (col)=w399) -> (element=w389:string)
            n147 = Or(x=w396, y=w395) -> (x .or. y?=w392:bool)
            n148 = Empty String/Path?(string/path=w389) -> (empty?=w393:bool)
            n149 = Or(x=w392, y=w393) -> (x .or. y?=w391:bool)
            n150 = case shown="False" w391 {
              tunnel: w390 -> [w413 _]
              tunnel: w389 -> [w412 _]
              tunnel: w387 -> [w408 _]
              tunnel: w386 -> [w407 _]
              tunnel: [w406 _] -> w385
              tunnel: w384 -> [w405 _]
              tunnel: w383 -> [w404 _]
              frame False {
                n151 = call-dynamic "get channels.vi"("module configuration in"=w413) -> ("channels"=w411:refnum<class "TBM channel.lvclass">[])  [unwired: 9 in, 1 out]
                n152 = call <vilib>:"find tag by name.vi"("name"=w412, "tags in"=w411) -> ("index"=w410:i32)  [unwired: 9 in]
                n153 = Index Array(array=w411, index=w410) -> (element=w409:refnum<class "TBM channel.lvclass">)
                n154 = case shown="0.." w410 {
                  tunnel: w409 -> [_ w424]
                  tunnel: w408 -> [_ w425]
                  tunnel: w407 -> [_ w423]
                  tunnel: [_ w416] -> w406
                  tunnel: w405 -> [_ w415]
                  tunnel: w404 -> [_ w414]
                  frame ..-1 {
                  }
                  frame 0.. {
                    n155 = call <vilib>:"find tag mapped to channel.vi"("owner"=w423, "channel"=w424, "engine configuration in"=w425) -> ("error out"=w420:errorcluster, "tag"=w422:refnum<class "tag descriptor.lvclass">, "engine configuration out"=w421:refnum<class "engine configuration.lvclass">)  [unwired: 6 in]
                    n156 = call-dynamic "get channels mapped to tag.vi"("error in"=w420, "tag"=w422, "engine configuration in"=w421) -> ("error out"=w419:errorcluster, "readers"=w417:T15[], "writer"=w418:T15)  [unwired: 5 in, 1 out]
                    n157 = case shown="No Error" w419 {
                      selector: w419 -> [_ w442]
                      tunnel: w418 -> [_ _]
                      tunnel: w417 -> [w430 _]
                      tunnel: [w429 w442] -> w416
                      tunnel: w415 -> [w426 _]
                      tunnel: w414 -> [w427 _]
                      frame No Error {
                        n158 = for {
                          tunnel: w430 -> [w441] mode=indexing
                          tunnel: [w438] -> w428 mode=concatenating
                          tunnel: w427 -> [w437]
                          tunnel: w426 -> [w435]
                          w431 = ".." ("string")
                          n159 = Unbundle By Name(w441) -> ("module ID"=w433:string, "channel"=w440:string)
                          n160 = Search 1D Array(1D array=w437, element=w433) -> (index of element=w436:i32)  [unwired: 1 in]
                          n161 = Index Array(array=w435, index=w436) -> (element=w434:string)
                          n162 = Concatenate Strings(w434, w431) -> (w432:string)
                          n163 = Concatenate Strings(w431, w440) -> (w439:string)
                          n164 = Build Array(w432, w439) -> (w438:string[])
                        }
                        n165 = property on="channels from input" class="LstBox (strict)"("Item Names"=w428) -> (error out=w429:errorcluster)  [unwired: 2 in, 1 out]
                      }
                      frame Error {
                      }
                    }
                  }
                }
              }
              frame True {
                # "nothing valid selected"
              }
            }
          }
          event "outputs": Value Change {
            w462 = 1  # chan column
            n166 = event-data() -> ("CtlRef"=w464:refnum<vi>)  [unwired: 1 in]
            n167 = local read "Module to View"() -> (w461:u16)
            n168 = property class="Engine Parent Editor Node.lvcla"(reference=w451) -> (reference out=w443:refnum<data-value>, "Data Access:Engine Configuration"=w450:refnum<class "engine configuration.lvclass">)  [unwired: 1 in, 1 out]
            n169 = property class="MCListbox (strict)"(reference=w464) -> ("ItemNames"=w463:string[][])  [unwired: 1 in, 2 out]
            n170 = Index Array(array=w457, index=w461) -> (element=w460:refnum<class "TBM module configuration.lvclass">)
            n171 = call <vilib>:"Read UID.vi"("configuration in"=w460) -> ("error out"=w458:errorcluster, "instance id"=w449:string, "configuration out"=w453:refnum<class "TBM module configuration.lvclass">)  [unwired: 8 in]
            n172 = Empty String/Path?(string/path=w449) -> (empty?=w459:bool)
            n173 = Index Array(array=w463, index (row)="outputs", index (col)=w462) -> (element=w452:string)
            n174 = Or(x=w459, y=w458) -> (x .or. y?=w455:bool)
            n175 = Empty String/Path?(string/path=w452) -> (empty?=w456:bool)
            n176 = Or(x=w455, y=w456) -> (x .or. y?=w454:bool)
            n177 = case shown="False" w454 {
              tunnel: w453 -> [w475 _]
              tunnel: w452 -> [w474 _]
              tunnel: w450 -> [w470 _]
              tunnel: w449 -> [w469 _]
              tunnel: [w468 _] -> w448
              tunnel: w447 -> [w467 _]
              tunnel: w446 -> [w466 _]
              frame False {
                n178 = call-dynamic "get channels.vi"("module configuration in"=w475) -> ("channels"=w473:refnum<class "TBM channel.lvclass">[])  [unwired: 9 in, 1 out]
                n179 = call <vilib>:"find tag by name.vi"("name"=w474, "tags in"=w473) -> ("index"=w472:i32)  [unwired: 9 in]
                n180 = Index Array(array=w473, index=w472) -> (element=w471:refnum<class "TBM channel.lvclass">)
                n181 = case shown="0.." w472 {
                  tunnel: w471 -> [_ w486]
                  tunnel: w470 -> [_ w487]
                  tunnel: w469 -> [_ w485]
                  tunnel: [_ w478] -> w468
                  tunnel: w467 -> [_ w477]
                  tunnel: w466 -> [_ w476]
                  frame ..-1 {
                  }
                  frame 0.. {
                    n182 = call <vilib>:"find tag mapped to channel.vi"("owner"=w485, "channel"=w486, "engine configuration in"=w487) -> ("error out"=w482:errorcluster, "tag"=w484:refnum<class "tag descriptor.lvclass">, "engine configuration out"=w483:refnum<class "engine configuration.lvclass">)  [unwired: 6 in]
                    n183 = call-dynamic "get channels mapped to tag.vi"("error in"=w482, "tag"=w484, "engine configuration in"=w483) -> ("error out"=w481:errorcluster, "readers"=w479:T15[], "writer"=w480:T15)  [unwired: 5 in, 1 out]
                    n184 = case shown="No Error" w481 {
                      selector: w481 -> [_ w511]
                      tunnel: w480 -> [w496 _]
                      tunnel: w479 -> [w499 _]
                      tunnel: [w498 w511] -> w478
                      tunnel: w477 -> [w493 _]
                      tunnel: w476 -> [w492 _]
                      frame No Error {
                        n185 = Unbundle By Name(w496) -> ("module ID"=w494:string, "channel"=w489:string)
                        n186 = for {
                          tunnel: w499 -> [w510] mode=indexing
                          tunnel: [w507] -> w497 mode=concatenating
                          tunnel: w492 -> [w506]
                          tunnel: w493 -> [w504]
                          w500 = ".." ("string")
                          n187 = Unbundle By Name(w510) -> ("module ID"=w502:string, "channel"=w509:string)
                          n188 = Search 1D Array(1D array=w506, element=w502) -> (index of element=w505:i32)  [unwired: 1 in]
                          n189 = Index Array(array=w504, index=w505) -> (element=w503:string)
                          n190 = Concatenate Strings(w503, w500) -> (w501:string)
                          n191 = Concatenate Strings(w500, w509) -> (w508:string)
                          n192 = Build Array(w501, w508) -> (w507:string[])
                        }
                        n193 = Search 1D Array(1D array=w492, element=w494) -> (index of element=w495:i32)  [unwired: 1 in]
                        n194 = Index Array(array=w493, index=w495) -> (element=w491:string)
                        n195 = Concatenate Strings(w491, "/\n" ("string"), w489) -> (→"Writer Channel":string)
                        n196 = property on="channels reading tag to outout" class="LstBox (strict)"("Item Names"=w497) -> (error out=w498:errorcluster)  [unwired: 2 in, 1 out]
                      }
                      frame Error {
                      }
                    }
                  }
                }
              }
              frame True {
                # "nothing valid selected"
              }
            }
          }
          event "Module 1", "Module 1 Filter": Value Change {
            n197 = event-data() -> ()  [unwired: 1 in, 6 out]
            n198 = Index Array(array=w520, index="Module 1") -> (element=w524:refnum<class "TBM module configuration.lvclass">)
            n199 = call <vilib>:"Read UID.vi"("configuration in"=w524) -> ("error out"=w522:errorcluster, "instance id"=w521:string, "configuration out"=w518:refnum<class "TBM module configuration.lvclass">)  [unwired: 8 in]
            n200 = Build Array("Module 1 Filter") -> (w516:string[])
            n201 = Empty String/Path?(string/path=w521) -> (empty?=w523:bool)
            n202 = Or(x=w523, y=w522) -> (x .or. y?=w519:bool)
            n203 = case shown="False" w519 {
              tunnel: w518 -> [w532 _]
              tunnel: w516 -> [w531 _]
              tunnel: [w527 _] -> w515
              frame False {
                n204 = call-dynamic "get channels.vi"("module configuration in"=w532) -> ("channels"=w530:refnum<class "TBM channel.lvclass">[])  [unwired: 9 in, 1 out]
                n205 = call <vilib>:"filter tags by name.vi"("allowable patterns"=w531, "tags in"=w530) -> ("filtered tags"=w529:refnum<class "tag descriptor.lvclass">[])  [unwired: 9 in]
                n206 = for {
                  tunnel: w529 -> [w534] mode=indexing
                  tunnel: [w533] -> w528 mode=indexing
                  n207 = call <vilib>:"read tag name.vi"("system tag in"=w534) -> ("name"=w533:string)  [unwired: 8 in, 2 out]
                }
                n208 = property on="Module 1 Channels" class="LstBox (strict)"("Item Names"=w528, "EditRow"=0 ("Edit Row")) -> (error out=w527:errorcluster)  [unwired: 2 in, 1 out]
              }
              frame True {
              }
            }
          }
          event "Module 2", "Module 2 Filter": Value Change {
            n209 = event-data() -> ()  [unwired: 1 in, 6 out]
            n210 = Index Array(array=w543, index="Module 2") -> (element=w547:refnum<class "TBM module configuration.lvclass">)
            n211 = call <vilib>:"Read UID.vi"("configuration in"=w547) -> ("error out"=w545:errorcluster, "instance id"=w544:string, "configuration out"=w541:refnum<class "TBM module configuration.lvclass">)  [unwired: 8 in]
            n212 = Build Array("Module 2 Filter") -> (w540:string[])
            n213 = Empty String/Path?(string/path=w544) -> (empty?=w546:bool)
            n214 = Or(x=w546, y=w545) -> (x .or. y?=w542:bool)
            n215 = case shown="False" w542 {
              tunnel: w541 -> [w555 _]
              tunnel: w540 -> [w554 _]
              tunnel: [w550 _] -> w539
              frame False {
                n216 = call-dynamic "get channels.vi"("module configuration in"=w555) -> ("channels"=w553:refnum<class "TBM channel.lvclass">[])  [unwired: 9 in, 1 out]
                n217 = call <vilib>:"filter tags by name.vi"("allowable patterns"=w554, "tags in"=w553) -> ("filtered tags"=w552:refnum<class "tag descriptor.lvclass">[])  [unwired: 9 in]
                n218 = for {
                  tunnel: w552 -> [w557] mode=indexing
                  tunnel: [w556] -> w551 mode=indexing
                  n219 = call <vilib>:"read tag name.vi"("system tag in"=w557) -> ("name"=w556:string)  [unwired: 8 in, 2 out]
                }
                n220 = property on="Module 2 Channels" class="LstBox (strict)"("Item Names"=w551, "EditRow"=0 ("Edit Row")) -> (error out=w550:errorcluster)  [unwired: 2 in, 1 out]
              }
              frame True {
              }
            }
          }
          event "attempt mapping": Value Change {
            n221 = event-data() -> ()  [unwired: 1 in, 1 out]
            n222 = local read "Module 1"() -> (w567:u16)
            n223 = local read "Module 2"() -> (w566:u16)
            n224 = property on="Module 2 Channels" class="LstBox (strict)"() -> ("Item Names"=w581:string[])  [unwired: 2 in, 2 out]
            n225 = property on="Module 1 Channels" class="LstBox (strict)"() -> ("Item Names"=w580:string[])  [unwired: 2 in, 2 out]
            n226 = Array Size(array="Module 1 Channels") -> (size(s)=w579:i32)
            n227 = Array Size(array="Module 2 Channels") -> (size(s)=w585:i32)
            n228 = Index Array(array=w568, index=w566) -> (element=w569:refnum<class "TBM module configuration.lvclass">)
            n229 = Index Array(array=w568, index=w567) -> (element=w576:refnum<class "TBM module configuration.lvclass">)
            n230 = Equal?(x=w579, y=w585) -> (x = y?=w578:bool)
            n231 = call <vilib>:"Read UID.vi"("configuration in"=w569) -> ("error out"=w571:errorcluster, "instance id"=w572:string, "configuration out"=w562:refnum<class "TBM module configuration.lvclass">)  [unwired: 8 in]
            n232 = call <vilib>:"Read UID.vi"("configuration in"=w576) -> ("error out"=w574:errorcluster, "instance id"=w573:string, "configuration out"=w563:refnum<class "TBM module configuration.lvclass">)  [unwired: 8 in]
            n233 = Empty String/Path?(string/path=w572) -> (empty?=w570:bool)
            n234 = Empty String/Path?(string/path=w573) -> (empty?=w575:bool)
            n235 = Or(x=w570, y=w571) -> (x .or. y?=w565:bool)
            n236 = Or(x=w575, y=w574) -> (x .or. y?=w564:bool)
            n237 = Compound Arithmetic op=AND(invert w564, invert w565, w578) -> (w577:bool)
            n238 = case shown="True" w577 {
              selector: w577 -> [w587 _]
              tunnel: [w587 TRUE] -> w584
              tunnel: "Module 2 Channels" -> [_ w606]
              tunnel: "Module 1 Channels" -> [_ w608]
              tunnel: w581 -> [_ w607]
              tunnel: w580 -> [_ w609]
              tunnel: w579 -> [_ w605]
              tunnel: w563 -> [_ w604]
              tunnel: w562 -> [_ w603]
              tunnel: w561 -> [_ w588]
              tunnel: [_ w595] -> w560
              frame False {
              }
              frame True {
                n239 = case shown="1.." w605 {
                  tunnel: w609 -> [w640 w646]
                  tunnel: w608 -> [_ w645]
                  tunnel: w607 -> [w639 w644]
                  tunnel: w606 -> [_ w643]
                  tunnel: [w640 w642] -> w599
                  tunnel: [w639 w641] -> w600
                  frame ..0 {
                  }
                  frame 1.. {
                    n240 = for {
                      tunnel: w644 -> [w649]
                      tunnel: w643 -> [w648] mode=indexing
                      tunnel: [w647] -> w641 mode=indexing
                      n241 = Index Array(array=w649, index=w648) -> (element=w647:string)
                    }
                    n242 = for {
                      tunnel: w646 -> [w652]
                      tunnel: w645 -> [w651] mode=indexing
                      tunnel: [w650] -> w642 mode=indexing
                      n243 = Index Array(array=w652, index=w651) -> (element=w650:string)
                    }
                  }
                }
                n244 = call-dynamic "get channels.vi"("module configuration in"=w604) -> ("channels"=w602:refnum<class "TBM channel.lvclass">[], "module configuration out"=w592:refnum<class "TBM module configuration.lvclass">)  [unwired: 9 in]
                n245 = call-dynamic "get channels.vi"("module configuration in"=w603) -> ("channels"=w601:refnum<class "TBM channel.lvclass">[], "module configuration out"=w590:refnum<class "TBM module configuration.lvclass">)  [unwired: 9 in]
                n246 = call <vilib>:"Read UID.vi"("configuration in"=w590) -> ("instance id"=w589:string)  [unwired: 8 in, 2 out]
                n247 = call <vilib>:"Read UID.vi"("configuration in"=w592) -> ("instance id"=w591:string)  [unwired: 8 in, 2 out]
                n248 = for {
                  tunnel: w601 -> [w632]
                  tunnel: w600 -> [w634] mode=indexing
                  tunnel: [w631] -> w594 mode=indexing
                  n249 = call <vilib>:"find tag by name.vi"("name"=w634, "tags in"=w632) -> ("index"=w633:i32)  [unwired: 9 in]
                  n250 = Index Array(array=w632, index=w633) -> (element=w631:refnum<class "TBM channel.lvclass">)
                }
                n251 = for {
                  tunnel: w602 -> [w637]
                  tunnel: w599 -> [w638] mode=indexing
                  tunnel: [w635] -> w593 mode=indexing
                  n252 = call <vilib>:"find tag by name.vi"("name"=w638, "tags in"=w637) -> ("index"=w636:i32)  [unwired: 9 in]
                  n253 = Index Array(array=w637, index=w636) -> (element=w635:refnum<class "TBM channel.lvclass">)
                }
                n254 = in-place {
                  in-place-border: [w621] -> w597
                  in-place-border: w594 -> [w613]
                  in-place-border: w593 -> [w612]
                  in-place-border: w591 -> [w611]
                  in-place-border: w589 -> [w610]
                  n255 = in-place-dvr #3(w588) -> (w618:refnum<class "Engine Parent Editor Node.lvclass">, w619:errorcluster)
                  n256 = call "read engine configuration.vi"("error in"=w619, "Engine Parent Editor Node in"=w618) -> ("error out"=w616:errorcluster, "engine configuration"=w615:refnum<class "engine configuration.lvclass">, "Engine Parent Editor Node out"=w617:refnum<class "Engine Parent Editor Node.lvclass">)  [unwired: 7 in]
                  n257 = for {
                    shift-right: [w627] -> w622
                    shift-left: w616 -> [w630]
                    shift-right: [w629] -> w614
                    shift-left: w615 -> [w628]
                    tunnel: w613 -> [w626] mode=indexing
                    tunnel: w612 -> [w625] mode=indexing
                    tunnel: w611 -> [w624]
                    tunnel: w610 -> [w623]
                    stop <- w627 stop-if-true
                    n258 = call <vilib>:"map channels together.vi"("owner 2"=w623, "owner 1"=w624, "error in"=w630, "channel 2"=w626, "channel 1"=w625, "engine configuration"=w628) -> ("error out"=w627:errorcluster, "engine configuration out"=w629:refnum<class "engine configuration.lvclass">)  [unwired: 4 in]
                  }
                  n259 = call "write engine configuration.vi"("error in"=w622, "engine configuration"=w614, "Engine Parent Editor Node in"=w617) -> ("error out"=w621:errorcluster, "Engine Parent Editor Node out"=w620:refnum<class "Engine Parent Editor Node.lvclass">)  [unwired: 7 in]
                  n260 = in-place-dvr #3(w620) -> (w596:errorcluster)  [unwired: 1 out]
                }
                n261 = Merge Errors(w597, w596) -> (w595:errorcluster)
              }
            }
            n262 = Or(x=w558, y=w584) -> (x .or. y?=w586:bool)
          }
        }
        n263 = case shown="Error" w80 {
          selector: w80 -> [w87 w89]
          tunnel: [w87 errorcluster {"status"=FALSE, "code"=0, "source"=""} ("error IO")] -> w82
          frame No Error {
          }
          frame Error {
            n264 = call <vilib>:"Simple Error Handler.vi"("error in (no error)"=w89) -> ()  [unwired: 4 in, 5 out]
          }
        }
      }
      n265 = case shown="True" w53 {
        tunnel: w46 -> [_ w65]
        tunnel: w47 -> [_ w64]
        tunnel: [_ w63] -> _
        frame False {
        }
        frame True {
          n266 = Generate User Event(user event=w65, event data cluster=w64) -> (error out=w63:errorcluster)  [unwired: 2 in, 1 out]
        }
      }
    }
    frame Error {
    }
  }
  n267 = Unregister For Events(event registration refnum=w34, error in=w33) -> (error out=w19:errorcluster)
  n268 = call <vilib>:"Simple Error Handler.vi"("error in (no error)"=w19) -> ()  [unwired: 4 in, 5 out]
